vi "Close MeasurementLink Session.vi"(8 "error in":errorcluster, 9 "initialize and close session behavior":T1, 10 "session in":variant, 11 "session factory in":refnum<class "Session Factory.lvclass">) -> (0 "error out":errorcluster)   [LabVIEW 2021, in "Session Management niSwitch.lvlib" / "Session Factory.lvclass"]
doc: "Closes the local session. If the session represents a remote session, <b>initialize and close session behavior</b> determines whether closing the local session closes the server session or detaches from the server session."
uses:
  Session Factory.lvclass
  <vilib>/Plug-In SDKs/Sessions/Instrument/ISession Factory/Initialize and Close Session Behavior.ctl
  NI Switch Client/RPC Messages/niswitch_grpc_CloseRequest.ctl
  NI Switch Client/RPC Messages/nidevice_grpc_Session.ctl
  NI Switch Client/RPC Messages/nidevice_grpc_Session_session/nidevice_grpc_Session_session.lvclass
  Session Factory.lvclass/Session Factory.ctl
  NI Switch Client/NI Switch Client.lvlib
  <vilib>/Plug-In SDKs/Sessions/Instrument/ISession Factory/ISession Factory.lvclass
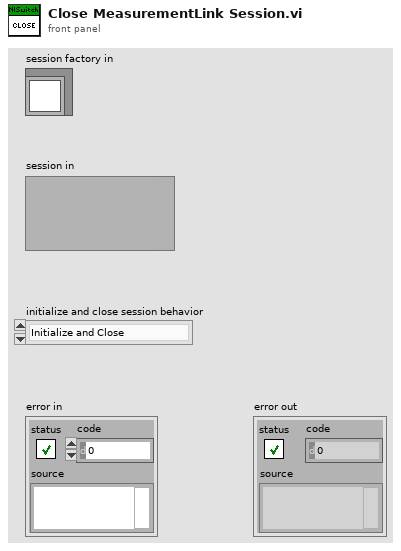
[diagram p1: front panel]
types:
  T1 = typedef "NI Session Management Instrument.lvlib/ISession Factory.lvclass/Initialize and Close Session Behavior.ctl" = enum16{"Initialize and Close", "Attach and Detach", "Initialize and Detach", "Attach and Close"}
  T2 = typedef "NI Switch Client.lvlib/niswitch_grpc_CloseRequest.ctl" = cluster{"vi":T3}
  T3 = typedef "NI Switch Client.lvlib/nidevice_grpc_Session.ctl" = cluster{"nidevice_grpc_Session_session":refnum<class "nidevice_grpc_Session_session.lvclass">}
  T4 = typedef "grpc-lvsupport-release.lvlib/grpcId.ctl" = u64
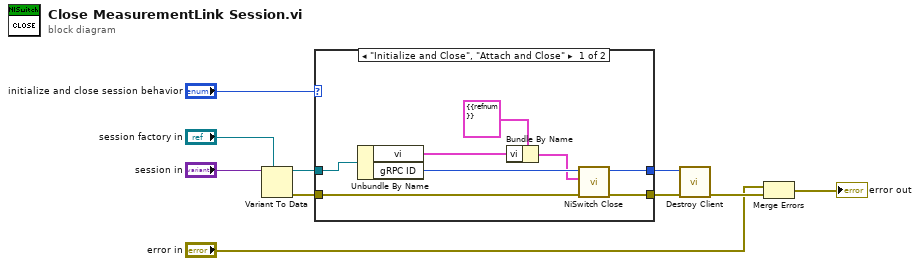
[diagram p0: block diagram]
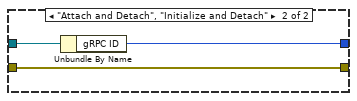
[diagram p2: hidden frame]
diagram:
  n1 = Variant To Data(type="session factory in", Variant="session in") -> (data=w5:refnum<class "Session Factory.lvclass">, error out=w7:errorcluster)  [unwired: 1 in]
  n2 = case shown="\"Initialize and Close\", \"Attach and Close\"" "initialize and close session behavior" {
    tunnel: [w11 w21] -> w4
    tunnel: w7 -> [w18 w21]
    tunnel: [w17 w20] -> w6
    tunnel: w5 -> [w16 w19]
    frame "Initialize and Close", "Attach and Close" {
      n3 = Unbundle By Name(w16) -> ("vi"=w14:T3, "gRPC ID"=w15:T4)
      n4 = Bundle By Name(cluster=T2 {"vi"={"nidevice_grpc_Session_session"=refnum}} ("Request Data"), "vi"=w14) -> (w12:T2)
      n5 = call "NiSwitch Close.vi"("error in"=w18, "Request Data"=w12, "gRPC ID"=w15) -> ("error out"=w11:errorcluster, "gRPC ID out"=w17:T4)  [unwired: 6 in, 1 out]
    }
    frame "Attach and Detach", "Initialize and Detach" {
      n6 = Unbundle By Name(w19) -> ("gRPC ID"=w20:T4)
    }
  }
  n7 = call "Destroy Client.vi"("error in"=w4, "gRPC ID"=w6) -> ("error out"=w3:errorcluster)  [unwired: 9 in]
  n8 = Merge Errors("error in", w3) -> (→"error out":errorcluster)
